vi "VM Spy - destroy variables.vi"(10 "Var Names":string[](array[string]), 11 "VC Handle":T1=-1) -> (0 "update":bool)   [LabVIEW 2021]
doc: "::: CalcExpress Toolkit :::\nCopyright (c) 2000-2026 Konstantin Shifershteyn. All rights reserved."
uses:
  vi.lib/addons/CalcExpress/cetypes.llb/VarMan Variable Context Handle.ctl
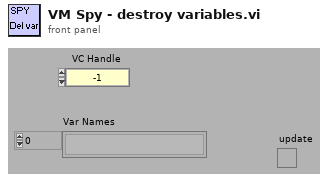
[diagram p1: front panel]
types:
  T1 = typedef "VarMan Variable Context Handle.ctl" = i32
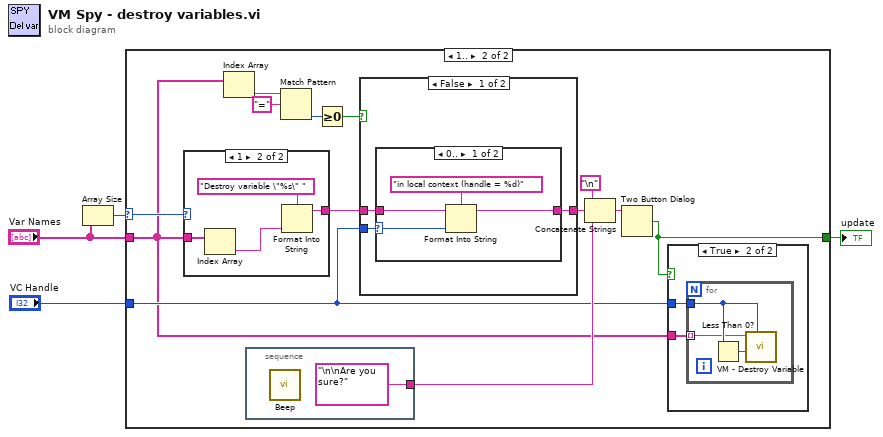
[diagram p0: block diagram]
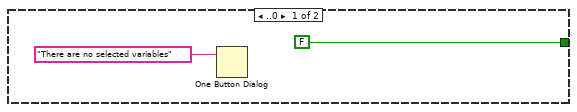
[diagram p2: hidden frame]
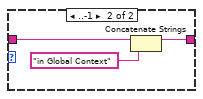
[diagram p3: hidden frame]
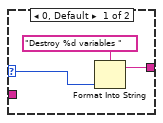
[diagram p5: hidden frame]
diagram:
  n1 = Array Size(array="Var Names") -> (size(s)=w4:i32)
  n2 = case shown="1.." w4 {
    selector: w4 -> [_ w14]
    tunnel: "VC Handle" -> [_ w16]
    tunnel: [FALSE ("T button?") w15] -> w2
    tunnel: "Var Names" -> [_ w12]
    frame ..0 {
      n3 = One Button Dialog(message="There are no selected variables") -> ()  [unwired: 1 in, 1 out]
    }
    frame 1.. {
      n4 = case shown="1" w14 {
        selector: w14 -> [w33 _]
        tunnel: w12 -> [_ w38]
        tunnel: [w34 w36] -> w13
        frame 0, Default {
          n5 = Format Into String(format string="Destroy %d variables ", w33) -> (resulting string=w34:string)  [unwired: 2 in, 1 out]
        }
        frame 1 {
          n6 = Index Array(array=w38) -> (element=w35:string)  [unwired: 1 in]
          n7 = Format Into String(format string="Destroy variable \"%s\" ", w35) -> (resulting string=w36:string)  [unwired: 2 in, 1 out]
        }
      }
      n8 = Index Array(array=w12) -> (element=w11:string)  [unwired: 1 in]
      n9 = stacked-sequence {
        tunnel: ["\n\nAre you sure?"] -> w19
        frame #0 {
          n10 = call <vilib>:"Beep.vi"() -> ()  [unwired: 12 in]
        }
      }
      n11 = Match Pattern(string=w11, regular expression="=") -> (offset past match=w9:i32)  [unwired: 1 in, 3 out]
      n12 = Greater Or Equal To 0?(x=w9) -> (x >= 0?=w8:bool)
      n13 = case shown="False" w8 {
        tunnel: [w23 w31] -> w18
        tunnel: w16 -> [w22 _]
        tunnel: w13 -> [w21 w31]
        frame False {
          n14 = case shown="0.." w22 {
            selector: w22 -> [w27 _]
            tunnel: [w25 w30] -> w23
            tunnel: w21 -> [w24 w28]
            frame 0.. {
              n15 = Format Into String(format string="in local context (handle = %d)", initial string=w24, w27) -> (resulting string=w25:string)  [unwired: 1 in, 1 out]
            }
            frame ..-1 {
              n16 = Concatenate Strings(w28, "in Global Context") -> (w30:string)
            }
          }
        }
        frame True {
        }
      }
      n17 = Concatenate Strings("\n", w18, w19) -> (w17:string)
      n18 = Two Button Dialog(message=w17) -> (T button?=w15:bool)  [unwired: 2 in]
      n19 = case shown="True" w15 {
        tunnel: w12 -> [_ w40]
        tunnel: w16 -> [_ w39]
        frame False {
        }
        frame True {
          n20 = for {
            tunnel: w40 -> [w41] mode=indexing
            tunnel: w39 -> [w42]
            n21 = Less Than 0?(x=w42) -> (x < 0?=w43:bool)
            n22 = call "VM - Destroy Variable.vi"("VC Handle"=w42, "global ? (F)"=w43, "name_spec"=w41) -> ()  [unwired: 5 in, 4 out]
          }
        }
      }
    }
  }
  "update" <- w2
